vi "WPI_GyroRomiGetAngle.vi"(8 "error in":errorcluster, 11 "GyroDevRef":T2={"DevStatus"={"status"=FALSE, "code"=0, "source"=""}, "Analog Channel"=enum."AI 1", "Gain (VoltsPerDegree/Second)"=0.0, "Gyro Type"=enum."Analog", "Handle"=0, "SPI Bus"=enum."Invalid", "Device Found"=FALSE, "Sample Rate"=1.0, "Calibrate On Open"=FALSE, "Offset"=0.0} {"Sample Rate" min=0.25 max=100.0 step=0.25}) -> (0 "error out":errorcluster, 1 "Anglular Rate":T1, 2 "Angle":T1, 3 "GyroDevRef":T2={"DevStatus"={"status"=FALSE, "code"=0, "source"=""}, "Analog Channel"=enum."AI 1", "Gain (VoltsPerDegree/Second)"=0.0, "Gyro Type"=enum."Analog", "Handle"=0, "SPI Bus"=enum."Invalid", "Device Found"=FALSE, "Sample Rate"=1.0, "Calibrate On Open"=FALSE, "Offset"=0.0} {"Sample Rate" min=0.25 max=100.0 step=0.25}, 4 "Calibrated?":bool)   [LabVIEW 2023]
doc: "Returns the angle, in degrees from the original heading, that the robot is currently facing.\n\nThis software is licensed. Open the labview\\readme\\WPI Robotics Library Open Source License.txt file for more information."
uses:
  <vilib>/Rock Robotics/WPI/Simulation/Protocol/Devices/Gyro/Gyro Update Ops.ctl
  <vilib>/Rock Robotics/WPI/Gyro/WPI_GyroDevRef.ctl
  <vilib>/Rock Robotics/SystemInterfaces/AI/FPGA_AIChannel.ctl
  <vilib>/Rock Robotics/SystemInterfaces/spilib/spi_bus.ctl
panel:
  # "Analog"
  # "XRS"
  # "Analog"
  # "XRS"
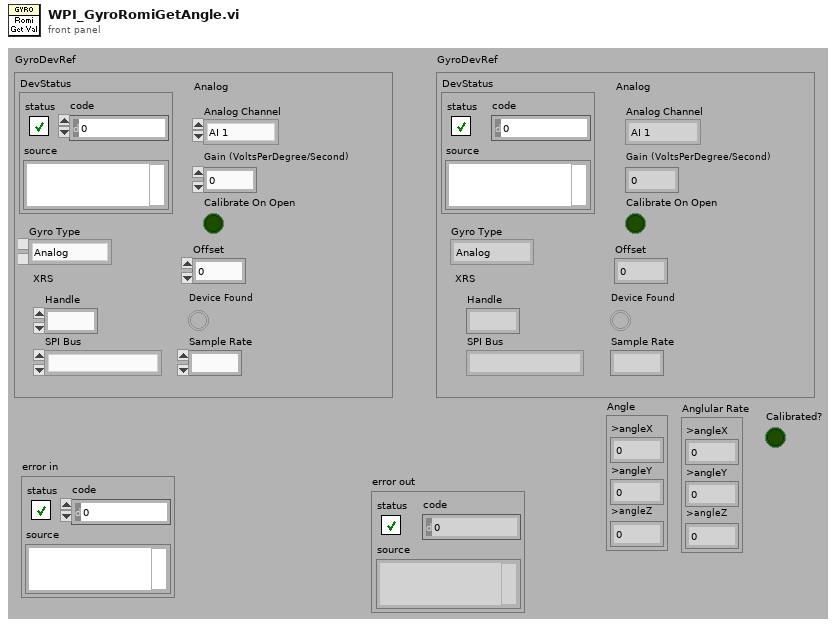
[diagram p1: front panel]
types:
  T1 = cluster{">angleX":dbl, ">angleY":dbl, ">angleZ":dbl}
  T2 = typedef "WPI_GyroDevRef.ctl" = cluster{"DevStatus":errorcluster, "Analog Channel":T3, "Gain (VoltsPerDegree/Second)":dbl, "Gyro Type":enum16{"Analog", "XRS450"}, "Handle":i32, "SPI Bus":T4, "Device Found":bool, "Sample Rate":dbl, "Calibrate On Open":bool, "Offset":dbl}
  T3 = typedef "FPGA_AIChannel.ctl" = enum8{"AI 0", "AI 1", "AI 2", "AI 3", "AI MXP 0", "AI MXP 1", "AI MXP 2", "AI MXP 3", "Invalid"}
  T4 = typedef "spi_bus.ctl" = enum16{"SPI On-Board, CS0", "SPI On-Board, CS1", "SPI On-Board, CS2", "SPI On-Board, CS3", "SPI MXP", "Invalid"}
  T5 = typedef "Gyro Update Ops.ctl" = enum16{"get", "delete", "JSON update", "set  name", "transmit initial", "reset", "set init", "set offsetX", "set offsetY", "set offsetZ", "set gain"}
  T6 = typedef "Gyro proto.ctl" = cluster{"type":string, "device":string, "name":string, "data":T7}
  T7 = typedef "Gyro Data proto.ctl" = cluster{"<init":bool, ">connected":bool, "<offsetX":dbl, "<offsetY":dbl, "<offsetZ":dbl, ">angleX":dbl, ">angleY":dbl, ">angleZ":dbl, ">rateX":dbl, ">rateY":dbl, ">rateZ":dbl, "<gain":dbl}
  T8 = cluster{"<offsetX":dbl, "<offsetY":dbl, "<offsetZ":dbl}
  T9 = cluster{">rateX":dbl, ">rateY":dbl, ">rateZ":dbl}
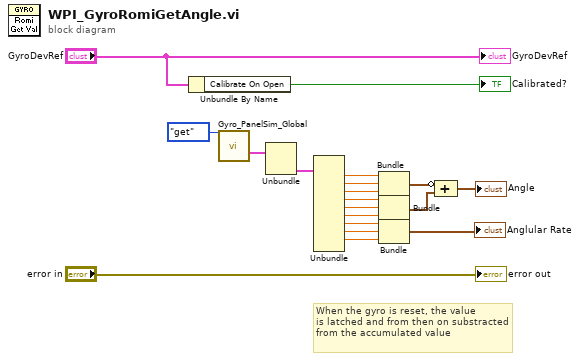
[diagram p0: block diagram]
diagram:
  # "When the gyro is reset, the value\nis latched and from then on substracted\nfrom the accumulated value"
  n1 = Unbundle By Name("GyroDevRef") -> ("Calibrate On Open"=→"Calibrated?":bool)
  n2 = call <vilib>:"Gyro_PanelSim_Global.vi"("Menu"=Gyro_Update_Ops."get") -> ("Value out"=w16:T6)  [unwired: 13 in, 1 out]
  n3 = Unbundle(w16) -> ("data"=w15:T7)  [unwired: 3 out]
  n4 = Unbundle(w15) -> ("<offsetX"=w4:dbl, "<offsetY"=w5:dbl, "<offsetZ"=w6:dbl, ">angleX"=w14:dbl, ">angleY"=w13:dbl, ">angleZ"=w12:dbl, ">rateX"=w11:dbl, ">rateY"=w10:dbl, ">rateZ"=w9:dbl)  [unwired: 3 out]
  n5 = Bundle("<offsetX"=w4, "<offsetY"=w5, "<offsetZ"=w6) -> (w3:T8)  [unwired: 1 in]
  n6 = Bundle(">angleX"=w14, ">angleY"=w13, ">angleZ"=w12) -> (w2:T1)  [unwired: 1 in]
  n7 = Bundle(">rateX"=w11, ">rateY"=w10, ">rateZ"=w9) -> (→"Anglular Rate":T9)  [unwired: 1 in]
  n8 = Compound Arithmetic op=ADD(invert w3, w2) -> (→"Angle":cluster{dbl, dbl, dbl})
  "GyroDevRef" <- "GyroDevRef"
  "error out" <- "error in"
